vi "Signal Profile selection.vi"(8 "Signal Tag A":string[](array[string]), 11 "Signal Profile Table A":string[][](table) caption="Singla Profile Table") -> (0 "Direction":string[](array[string]), 1 "Seq ENo":string[](array[string]), 2 "Mx Right No":string[](array[string]), 3 "Seq SNo":string[](array[string]), 4 "File name":string[](array[string]), 5 "S IDX":string[](array[string]), 6 "Mx Right Read Seq":string[](array[string]))   [LabVIEW 2018]
panel:
  out "サイズ":i32
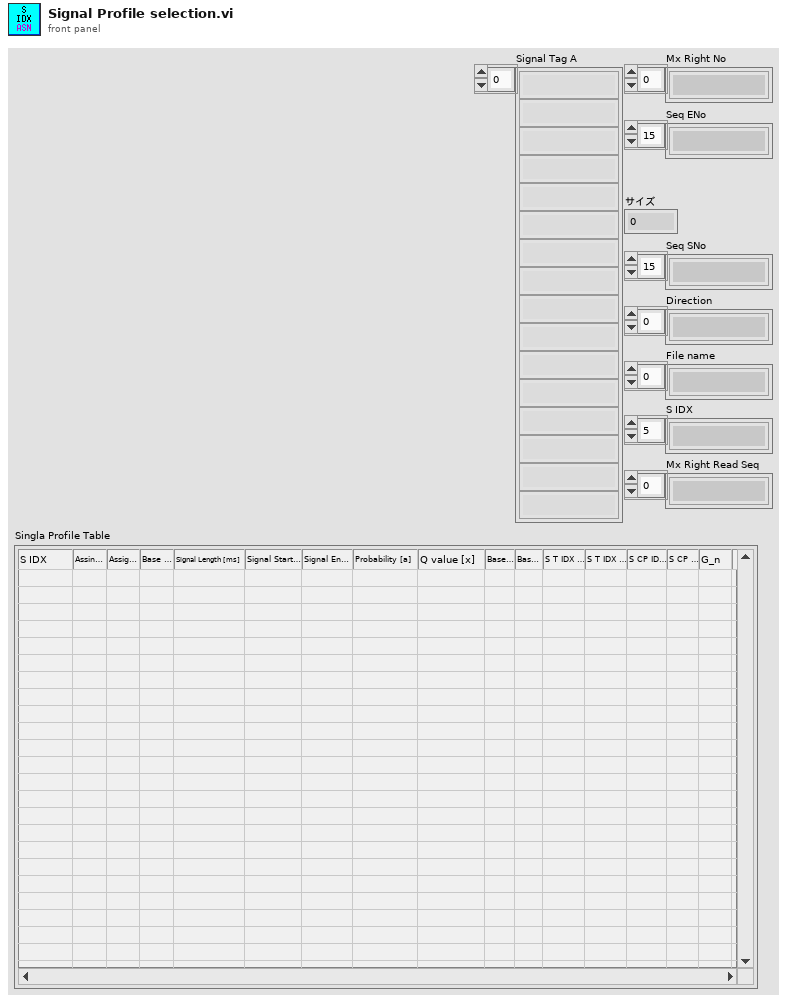
[diagram p1: front panel]
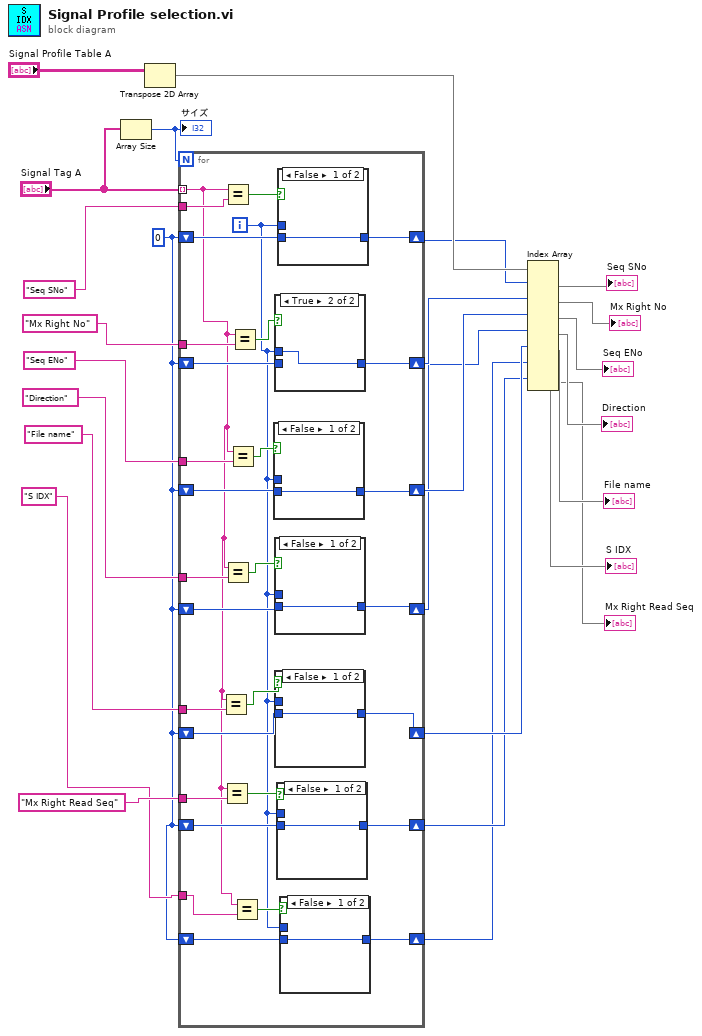
[diagram p0: block diagram]
diagram:
  w2 = 0
  n1 = Array Size(array="Signal Tag A") -> (size(s)=w26:i32)
  "サイズ" <- w26
  n2 = Transpose 2D Array(2D array="Signal Profile Table A") -> (transposed array=w22:string[][])
  n3 = for {
    N: w26 -> [_]
    tunnel: "Signal Tag A" -> [w31] mode=indexing
    tunnel: "Seq SNo" -> [w56]
    shift-right: [w54] -> w20
    shift-left: w2 -> [w55]
    shift-right: [w51] -> w19
    shift-left: w2 -> [w52]
    shift-right: [w49] -> w17
    shift-left: w2 -> [w50]
    shift-right: [w47] -> w15
    shift-left: w2 -> [w48]
    shift-right: [w45] -> w13
    shift-left: w2 -> [w46]
    tunnel: "Mx Right No" -> [w43]
    tunnel: "Seq ENo" -> [w42]
    tunnel: "Direction" -> [w41]
    tunnel: "File name" -> [w40]
    shift-right: [w35] -> w5
    shift-left: w2 -> [w36]
    tunnel: "Mx Right Read Seq" -> [w33]
    tunnel: "S IDX" -> [w30]
    shift-right: [w27] -> w1
    shift-left: w2 -> [w28]
    i -> [w29]
    n4 = Equal?(x=w31, y=w40) -> (x = y?=w37:bool)
    n5 = Equal?(x=w31, y=w33) -> (x = y?=w34:bool)
    n6 = Equal?(x=w31, y=w56) -> (x = y?=w53:bool)
    n7 = Equal?(x=w31, y=w41) -> (x = y?=w38:bool)
    n8 = Equal?(x=w31, y=w42) -> (x = y?=w39:bool)
    n9 = Equal?(x=w31, y=w43) -> (x = y?=w44:bool)
    n10 = Equal?(x=w31, y=w30) -> (x = y?=w32:bool)
    n11 = case shown="False" w39 {
      tunnel: w29 -> [_ w66]
      tunnel: [w65 w66] -> w49
      tunnel: w50 -> [w65 _]
      frame False {
      }
      frame True {
      }
    }
    n12 = case shown="True" w44 {
      tunnel: w29 -> [_ w68]
      tunnel: [w67 w68] -> w51
      tunnel: w52 -> [w67 _]
      frame False {
      }
      frame True {
      }
    }
    n13 = case shown="False" w38 {
      tunnel: w29 -> [_ w64]
      tunnel: [w63 w64] -> w47
      tunnel: w48 -> [w63 _]
      frame False {
      }
      frame True {
      }
    }
    n14 = case shown="False" w37 {
      tunnel: w29 -> [_ w62]
      tunnel: [w61 w62] -> w45
      tunnel: w46 -> [w61 _]
      frame False {
      }
      frame True {
      }
    }
    n15 = case shown="False" w34 {
      tunnel: w29 -> [_ w60]
      tunnel: [w59 w60] -> w35
      tunnel: w36 -> [w59 _]
      frame False {
      }
      frame True {
      }
    }
    n16 = case shown="False" w53 {
      tunnel: w29 -> [_ w70]
      tunnel: [w69 w70] -> w54
      tunnel: w55 -> [w69 _]
      frame False {
      }
      frame True {
      }
    }
    n17 = case shown="False" w32 {
      tunnel: w29 -> [_ w58]
      tunnel: [w57 w58] -> w27
      tunnel: w28 -> [w57 _]
      frame False {
      }
      frame True {
      }
    }
  }
  n18 = Index Array(array=w22, index (row) #1=w20, index (row) #2=w19, index (row) #3=w17, index (row) #4=w15, index (row) #5=w13, index (row) #6=w1, index (row) #7=w5) -> (element #1=→"Seq SNo":string[], element #2=→"Mx Right No":string[], element #3=→"Seq ENo":string[], element #4=→"Direction":string[], element #5=→"File name":string[], element #6=→"S IDX":string[], element #7=→"Mx Right Read Seq":string[])  [unwired: 7 in]
